vi "Header Cluster to XNET CAN.vi"(10 "TAI Time (ns)":i64, 11 "Socket CAN Header":T3 {"CANID and Flags" format="%.0x"; "FD Flags" format="%.0x"}) -> (3 "XNET CAN frame":T1 {"payload" format="%x"; "timestamp" format="%<%.7X\n%x>T"; "type" items=["CAN Data"=0, "CAN Remote"=1, "CAN Bus Error"=2, "CAN 2.0 Data"=8, "CAN FD Data"=16, "CAN FD+BRS Data"=24, "J1939 Data"=192, "Delay"=224, "Log Trigger"=225, "Start Trigger"=226]; "identifier" format="%x"}, 5 "Unsupported":bool)   [LabVIEW 2021, in "XNET CAN RW.lvclass"]
uses:
  XNET CAN RW.lvclass
  <vilib>/CIF Foundation/CIF PCAP Parse and Build/Typedef/Format Specific/Socket CAN Header.ctl
  <vilib>/xnet/xnet.llb/XNET Frame CAN.ctl
  <vilib>/xnet/xnet.llb/XNET Frame Type CAN.ctl
  XNET CAN RW.lvclass/XNET CAN RW.ctl
  <vilib>/CIF Foundation/CIF Utilities/Time/Time_CIF_U.lvlib
  <vilib>/CIF Foundation/CIF PCAP Parse and Build/pcap_Parse_Build_CIF.lvclass
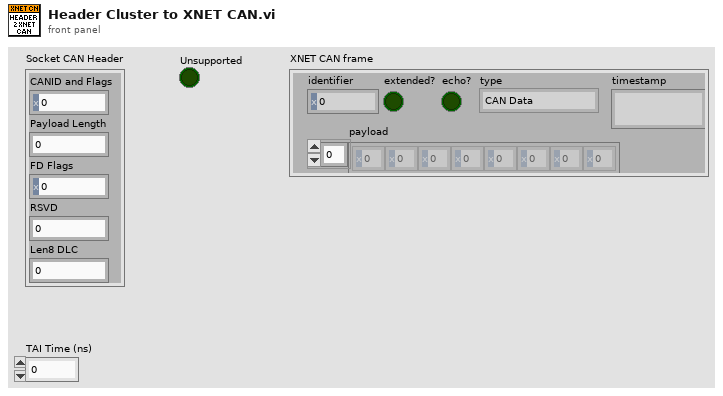
[diagram p1: front panel]
types:
  T1 = typedef "XNET Frame CAN.ctl" = cluster{"timestamp":timestamp, "payload":u8[], "identifier":u32, "type":T2, "extended?":bool, "echo?":bool}
  T2 = typedef "XNET Frame Type CAN.ctl" = u8
  T3 = typedef "pcap_Parse_Build_CIF.lvclass/Socket CAN Header.ctl" = cluster{"CANID and Flags":u32, "Payload Length":u8, "FD Flags":u8, "RSVD":u8, "Len8 DLC":u8}
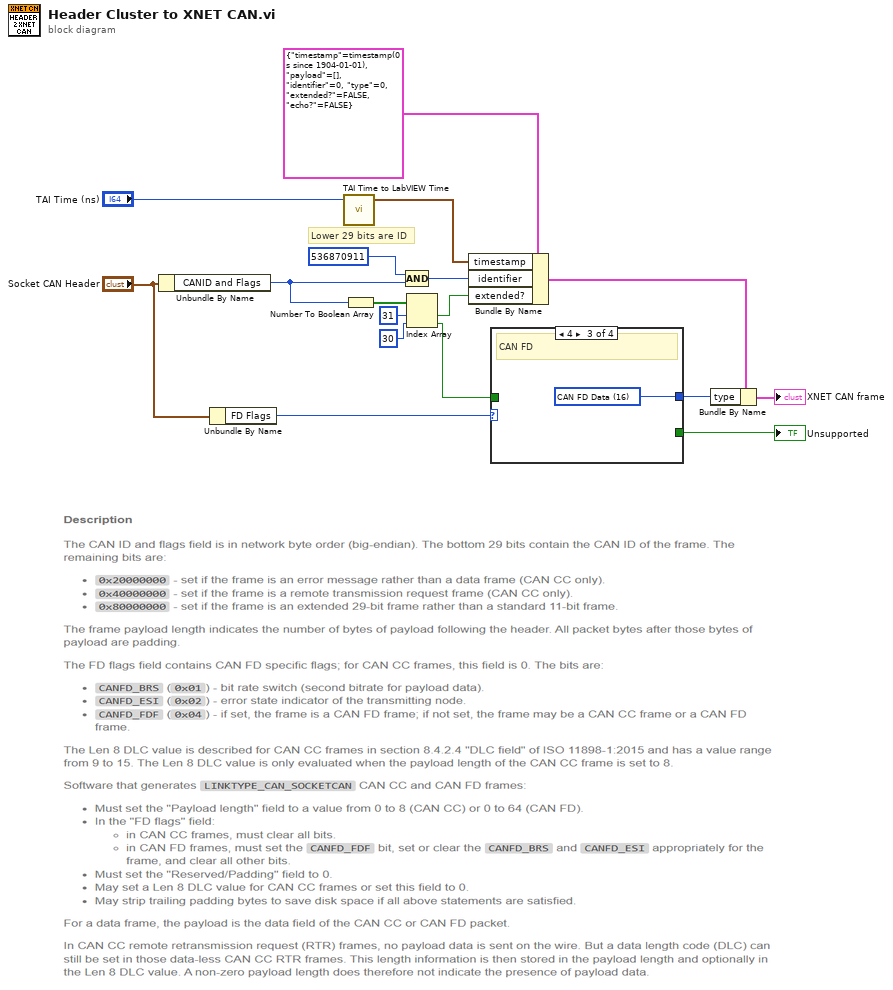
[diagram p0: block diagram]
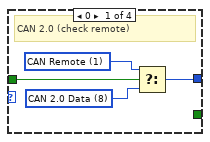
[diagram p2: hidden frame]
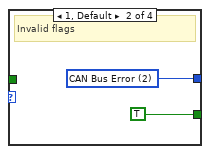
[diagram p3: hidden frame]
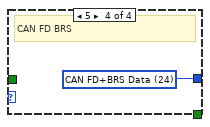
[diagram p4: hidden frame]
diagram:
  # "Lower 29 bits are ID"
  n1 = Unbundle By Name("Socket CAN Header") -> ("CANID and Flags"=w15:u32)
  n2 = Unbundle By Name("Socket CAN Header") -> ("FD Flags"=w8:u8)
  n3 = call <vilib>:"TAI Time to LabVIEW Time.vi"("TAI Time (ns)"="TAI Time (ns)") -> ("LabVIEW Time (s)"=w10:timestamp)  [unwired: 4 in]
  n4 = Number To Boolean Array(number=w15) -> (Boolean array=w14:bool[])
  n5 = Compound Arithmetic op=AND(u32 536870911 ("number"), w15) -> (w16:u32)
  n6 = Index Array(array=w14, index #1=31 ("index"), index #2=30 ("index")) -> (element #1=w12:bool, element #2=w7:bool)
  n7 = Bundle By Name(cluster=T1 {"timestamp"=timestamp(0 s since 1904-01-01), "payload"=[], "identifier"=0, "type"=0, "extended?"=FALSE, "echo?"=FALSE} ("XNET CAN frame 2"), "timestamp"=w10, "identifier"=w16, "extended?"=w12) -> (w5:T1)
  n8 = case shown="4" w8 {
    tunnel: w7 -> [w21 _ _ _]
    tunnel: [w20 w22 w24 w25] -> w6
    tunnel: [_ TRUE _ _] -> w4
    frame 0 {
      w18 = T2 1 items=["CAN Data"=0, "CAN Remote"=1, "CAN Bus Error"=2, "CAN 2.0 Data"=8, "CAN FD Data"=16, "CAN FD+BRS Data"=24, "J1939 Data"=192, "Delay"=224, "Log Trigger"=225, "Start Trigger"=226] ("type")
      w19 = T2 8 items=["CAN Data"=0, "CAN Remote"=1, "CAN Bus Error"=2, "CAN 2.0 Data"=8, "CAN FD Data"=16, "CAN FD+BRS Data"=24, "J1939 Data"=192, "Delay"=224, "Log Trigger"=225, "Start Trigger"=226] ("type")
      # "CAN 2.0 (check remote)"
      n9 = Select(t=w18, s=w21, f=w19) -> (s? t:f=w20:T2)
    }
    frame 1, Default {
      w22 = T2 2 items=["CAN Data"=0, "CAN Remote"=1, "CAN Bus Error"=2, "CAN 2.0 Data"=8, "CAN FD Data"=16, "CAN FD+BRS Data"=24, "J1939 Data"=192, "Delay"=224, "Log Trigger"=225, "Start Trigger"=226] ("type")
      # "Invalid flags"
    }
    frame 4 {
      w24 = T2 16 items=["CAN Data"=0, "CAN Remote"=1, "CAN Bus Error"=2, "CAN 2.0 Data"=8, "CAN FD Data"=16, "CAN FD+BRS Data"=24, "J1939 Data"=192, "Delay"=224, "Log Trigger"=225, "Start Trigger"=226] ("type")
      # "CAN FD"
    }
    frame 5 {
      w25 = T2 24 items=["CAN Data"=0, "CAN Remote"=1, "CAN Bus Error"=2, "CAN 2.0 Data"=8, "CAN FD Data"=16, "CAN FD+BRS Data"=24, "J1939 Data"=192, "Delay"=224, "Log Trigger"=225, "Start Trigger"=226] ("type")
      # "CAN FD BRS"
    }
  }
  "Unsupported" <- w4
  n10 = Bundle By Name(cluster=w5, "type"=w6) -> (→"XNET CAN frame":T1)
